vi "OwnFile20261012_Native_GetSubVIPath.vi"() -> ()   [LabVIEW 2024]
panel:
  out "error out":errorcluster caption="错误输出"
  out "vi_path":path
  in  "subvi_id":u32
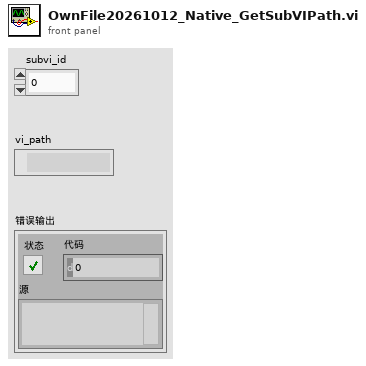
[diagram p1: front panel]
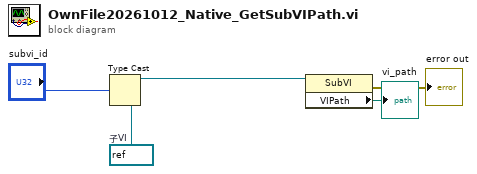
[diagram p0: block diagram]
diagram:
  w4 = refnum<vi> refnum  # 子VI
  n1 = Type Cast ("强制类型转换")(type=w4, x="subvi_id") -> (*(type *) &x=w3:refnum<vi>)
  n2 = property on="属性节点" class="SubVI"(reference=w3) -> (error out=→"error out":errorcluster, "VIPath"=→"vi_path":path)  [unwired: 1 in, 1 out]
